vi "RR Read number including repeat.vi"(8 "noise MAX":i32=3, 11 "RR Read No":i32[](array[numeric])) -> (0 "RR %":dbl[](array[numeric]), 1 "RR N#":i32[](array[numeric]), 2 "RR T#":i32, 3 "シグナル集計":dbl[][](array[numeric]), 4 "Average Read N":dbl format="%#_4g", 5 "最大値":i32, 6 "Av n#":dbl, 7 "Av RR n#bp":i32)   [LabVIEW 2018]
panel:
  out "S#":i32[](array[numeric])
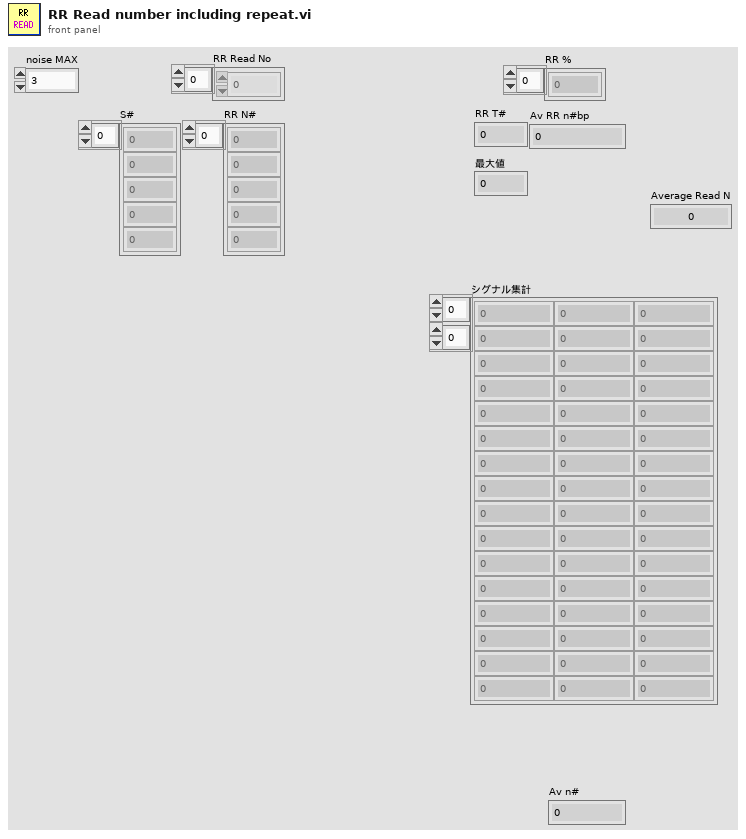
[diagram p1: front panel]
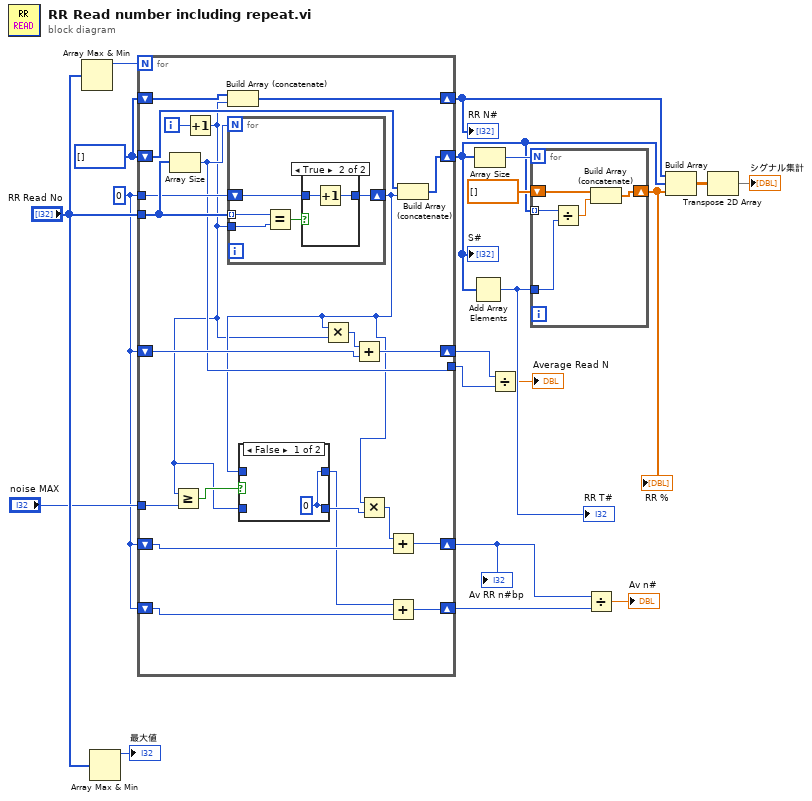
[diagram p0: block diagram]
diagram:
  w4 = 0
  w19 = i32[] []
  n1 = Array Max & Min(array="RR Read No") -> (max value=w20:i32)  [unwired: 3 out]
  n2 = Array Max & Min(array="RR Read No") -> (max value=→"最大値":i32)  [unwired: 3 out]
  n3 = for {
    N: w20 -> [_]
    tunnel: "RR Read No" -> [w42]
    tunnel: w4 -> [w40]
    shift-right: [w39] -> w12
    shift-left: w19 -> [w38]
    shift-right: [w37] -> w11
    shift-left: w19 -> [w36]
    shift-right: [w33] -> w8
    shift-left: w4 -> [w34]
    tunnel: [w30] -> w9
    tunnel: "noise MAX" -> [w32]
    shift-right: [w26] -> w2
    shift-left: w4 -> [w25]
    shift-right: [w24] -> w1
    shift-left: w4 -> [w23]
    i -> [w41]
    n4 = Array Size(array=w42) -> (size(s)=w30:i32)
    n5 = Increment(x=w41) -> (x+1=w21:i32)
    n6 = Greater Or Equal?(x=w21, y=w32) -> (x >= y?=w31:bool)
    n7 = Build Array (concatenate)(w36, w21) -> (w37:i32[])
    n8 = for {
      N: w30 -> [_]
      tunnel: w42 -> [w48] mode=indexing
      tunnel: w21 -> [w49]
      shift-right: [w46] -> w28
      shift-left: w40 -> [w47]
      n9 = Equal?(x=w48, y=w49) -> (x = y?=w50:bool)
      n10 = case shown="True" w50 {
        tunnel: [w51 w53] -> w46
        tunnel: w47 -> [w51 w52]
        frame False {
        }
        frame True {
          n11 = Increment(x=w52) -> (x+1=w53:i32)
        }
      }
    }
    n12 = case shown="False" w31 {
      tunnel: w21 -> [_ w45]
      tunnel: [w43 w45] -> w27
      tunnel: w28 -> [_ w44]
      tunnel: [w43 w44] -> w22
      frame False {
        w43 = 0
      }
      frame True {
      }
    }
    n13 = Multiply(x=w28, y=w21) -> (x*y=w35:i32)
    n14 = Add(x=w35, y=w34) -> (x+y=w33:i32)
    n15 = Multiply(x=w28, y=w27) -> (x*y=w29:i32)
    n16 = Add(x=w29, y=w25) -> (x+y=w26:i32)
    n17 = Add(x=w22, y=w23) -> (x+y=w24:i32)
    n18 = Build Array (concatenate)(w38, w28) -> (w39:i32[])
  }
  "S#" <- w12
  "RR N#" <- w11
  "Av RR n#bp" <- w2
  n19 = Add Array Elements(numeric array=w12) -> (sum=w18:i32)
  "RR T#" <- w18
  n20 = Array Size(array=w12) -> (size(s)=w17:i32)
  n21 = Divide(x=w8, y=w9) -> (x/y=→"Average Read N":dbl)
  n22 = for {
    N: w17 -> [_]
    tunnel: w12 -> [w58] mode=indexing
    tunnel: w18 -> [w57]
    shift-right: [w55] -> w13
    shift-left: dbl[] [] -> [w54]
    n23 = Divide(x=w58, y=w57) -> (x/y=w56:dbl)
    n24 = Build Array (concatenate)(w54, w56) -> (w55:dbl[])
  }
  "RR %" <- w13
  n25 = Divide(x=w2, y=w1) -> (x/y=→"Av n#":dbl)
  n26 = Build Array(w11, w12, w13) -> (w15:dbl[][])
  n27 = Transpose 2D Array(2D array=w15) -> (transposed array=→"シグナル集計":dbl[][])
